vi "Start Processes.vi"(8 "error in (no error)":errorcluster, 9 "Timeout [ms] (-1)":i32=-1, 11 "Application In":refnum<class "Application.lvclass">) -> (0 "error out":errorcluster, 3 "Application Out":refnum<class "Application.lvclass">)   [LabVIEW 2020, in "Application.lvclass"]
uses:
  Application.lvclass
  Application.lvclass/Application.ctl
  Process/Process.lvclass
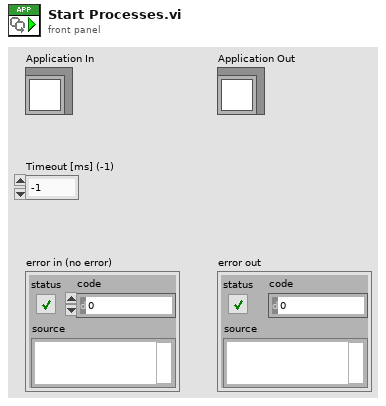
[diagram p1: front panel]
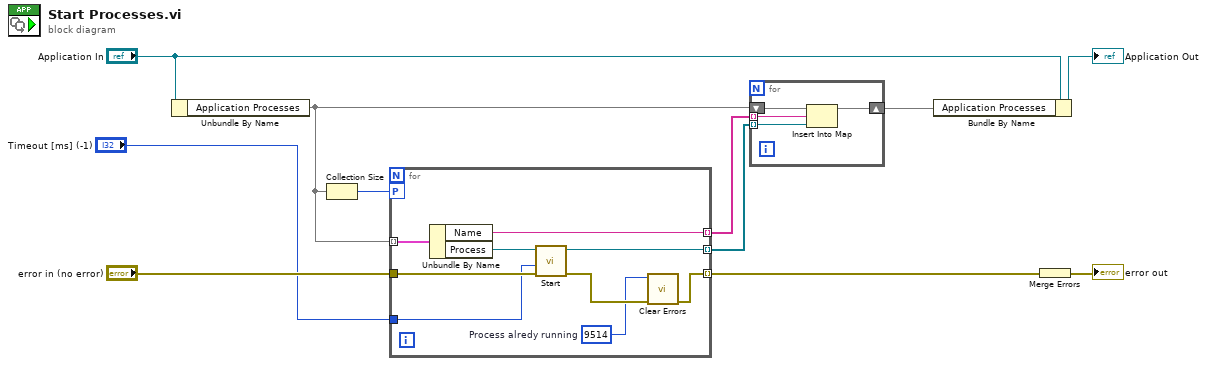
[diagram p0: block diagram]
diagram:
  n1 = Unbundle By Name("Application In") -> ("Application Processes"=w4:map{string, refnum<class "Process.lvclass">})
  n2 = Collection Size(1:w4) -> (0:w6:i32)
  n3 = for {
    tunnel: w4 -> [w18] mode=indexing
    tunnel: "error in (no error)" -> [w19]
    tunnel: [w13] -> w10 mode=indexing
    workers-P: w6 -> [_]
    tunnel: "Timeout [ms] (-1)" -> [w17]
    tunnel: [w16] -> w2 mode=indexing
    tunnel: [w15] -> w1 mode=indexing
    w12 = 9514  # Process alredy running
    n4 = Unbundle By Name(w18) -> ("Name"=w16:string, "Process"=w14:refnum<class "Process.lvclass">)
    n5 = call "Start.vi"("error in (no error)"=w19, "Timeout [ms] (-1)"=w17, "Process In"=w14) -> ("error out"=w20:errorcluster, "Process Out"=w15:refnum<class "Process.lvclass">)  [unwired: 6 in, 1 out]
    n6 = call <vilib>:"Clear Errors.vi"("error in (no error)"=w20, "specific error code to clear (0: all)"=w12) -> ("error out"=w13:errorcluster)  [unwired: 4 in, 1 out]
  }
  n7 = for {
    shift-right: [w23] -> w3
    shift-left: w4 -> [w24]
    tunnel: w2 -> [w22] mode=indexing
    tunnel: w1 -> [w21] mode=indexing
    n8 = Insert Into Map(map in=w24, key=w22, value=w21) -> (map out=w23:map{string, refnum<class "Process.lvclass">})  [unwired: 2 out]
  }
  n9 = Bundle By Name(cluster="Application In", "Application Processes"=w3) -> (→"Application Out":refnum<class "Application.lvclass">)
  n10 = Merge Errors(w10) -> (→"error out":errorcluster)
